vi "D+M Sense.vi"(8 "error in":errorcluster) -> (0 "error out":errorcluster, 2 "Result":string, 3 "RESULT":bool)   [LabVIEW 2021]
uses:
  DUT/DUT_Cmd.ctl
  10054_Control Folder/Support/10054_states.ctl
panel:
  out "Command Response 2":string
  out "number 2":dbl
  out "UnPlugged":bool
  out "Plugged":bool
  out "number":dbl
  out "Command Response":string
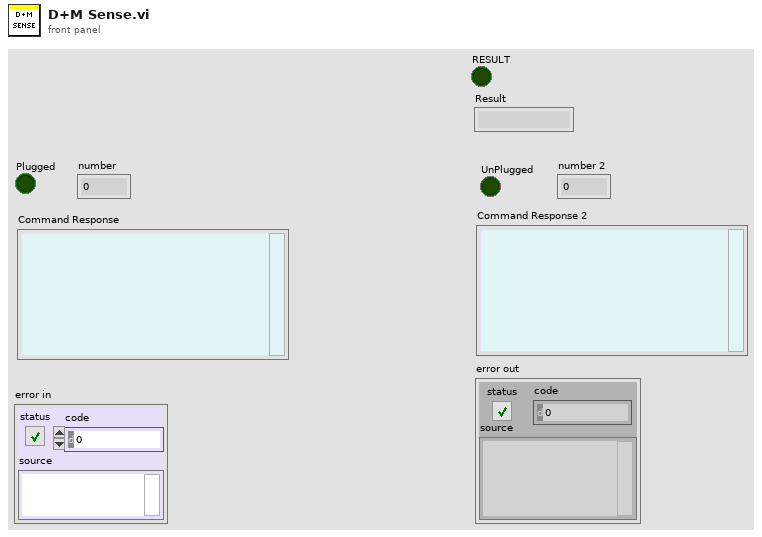
[diagram p1: front panel]
types:
  T1 = typedef "10054_states.ctl" = enum16{"Pilz-1", "Pilz-2", "AC CON - 2", "AC CON - 3", "AC CON - 4", "AC CON - 5", "Tower Lamp - Red", "Tower Lamp - Amber", "Tower Lamp - Green", "FAN 1 & 2", "FAN 3 & 4", "FAN 5 & 6", "Load - 1 10A", "Load - 2 10A", "Load - 3 5A", "Load - 4 5A", "Load - 5 2A", "TP49 - 12V", "TP20 - 5V", "TP148 - 3.3", "TP193 - GND", "J11.1 POS", "J11.2 NEG", "Noti LED POS", "Noti LED NEG", "Noti LED  5V", "D+M J14.1 - 3.3", "D+M J14.2 - GND", "NFC - 1", "NFC - 2"}
  T2 = typedef "DUT_Cmd.ctl" = enum16{"Unlock serial", "Stop console logs", "Release emergency at start", "Read firmware", "WiFi credentials", "WiFi connected", "WiFi SSID", "Board revision", "ADC_NTC_TEMP", "ADC_TYPE2_RCD_CURRENT", "PCBA serial write", "PCBA serial readback", "Start energy meter", "Energy meter Vac", "Energy meter Iac", "Energy meter PF", "Energy meter energy", "Provision", "Set gateway identity", "CP checklist", "Earth detect", "D+M sense unplugged", "D+M sense plugged", "Output relay weld", "Start diagnostics", "Relay 1 on", "Relay 2 on", "Emergency pressed", "Release emergency", "Emergency released", "Unlock serial for 5 A", "Board current (5 A)", "Unlock serial for 15 A", "Board current (15 A)", "Unlock serial for 0 A", "NFC tag", "Start diagnostics again", "Relay 2 off", "Relay 1 off", "End diagnostics", "Load current (5 A) [No USB station]", "Load current (15 A) [No USB station]", "Load current (0 A) [No USB station]", "NFC tag [No USB station]", "Battery Voltage", "FW Power reset", "Notification LED", "O/P Relay weld Detection", "Earth Detection", "12V ", "5V", "3.3V"}
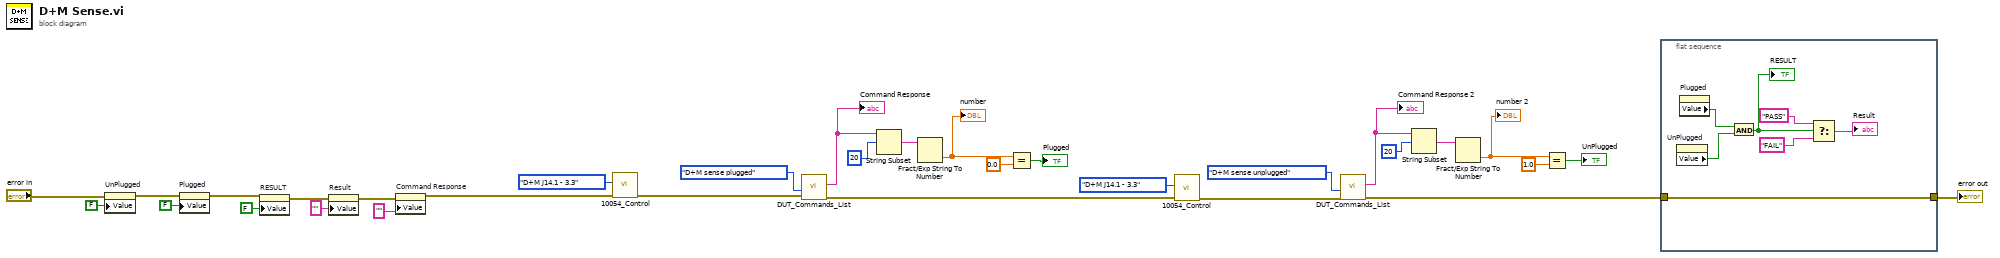
[diagram p0: block diagram]
diagram:
  n1 = property on="UnPlugged" class="Bool (strict)"(error in="error in", "Value"=FALSE ("UnPlugged")) -> (error out=w15:errorcluster)  [unwired: 1 in, 1 out]
  n2 = property on="Plugged" class="Bool (strict)"(error in=w15, "Value"=FALSE ("Plugged")) -> (error out=w14:errorcluster)  [unwired: 1 in, 1 out]
  n3 = property on="RESULT" class="Bool (strict)"(error in=w14, "Value"=FALSE ("RESULT")) -> (error out=w13:errorcluster)  [unwired: 1 in, 1 out]
  n4 = property on="Result" class="Str"(error in=w13, "Value"="" ("Result")) -> (error out=w12:errorcluster)  [unwired: 1 in, 1 out]
  n5 = property on="Command Response" class="Str"(error in=w12, "Value"="" ("Command Response")) -> (error out=w2:errorcluster)  [unwired: 1 in, 1 out]
  n6 = call "10054_Control.vi"("error in"=w2, "Pin"=10054_states."D+M J14.1 - 3.3") -> ("error out"=w1:errorcluster)  [unwired: 5 in, 3 out]
  n7 = call "DUT_Commands_List.vi"("error in"=w1, "DUT Cmd"=DUT_Cmd."D+M sense plugged") -> ("error out"=w6:errorcluster, "Command Response"=w30:string)  [unwired: 7 in, 1 out]
  "Command Response" <- w30
  n8 = String Subset(string=w30, offset (0)=20) -> (substring=w28:string)  [unwired: 1 in]
  n9 = Fract/Exp String To Number(string=w28) -> (number=w27:dbl)  [unwired: 3 in, 1 out]
  "number" <- w27
  n10 = Equal?(x=w27, y=0.0) -> (x = y?=→"Plugged":bool)
  n11 = call "10054_Control.vi"("error in"=w6, "Pin"=10054_states."D+M J14.1 - 3.3") -> ("error out"=w5:errorcluster)  [unwired: 5 in, 3 out]
  n12 = call "DUT_Commands_List.vi"("error in"=w5, "DUT Cmd"=DUT_Cmd."D+M sense unplugged") -> ("error out"=w17:errorcluster, "Command Response"=w19:string)  [unwired: 7 in, 1 out]
  "Command Response 2" <- w19
  n13 = String Subset(string=w19, offset (0)=20) -> (substring=w21:string)  [unwired: 1 in]
  n14 = Fract/Exp String To Number(string=w21) -> (number=w22:dbl)  [unwired: 3 in, 1 out]
  "number 2" <- w22
  n15 = Equal?(x=w22, y=1.0) -> (x = y?=→"UnPlugged":bool)
  n16 = flat-sequence {
    tunnel: w17 -> [w34]
    tunnel: [w34] -> w16
    frame #0 {
      n17 = property on="UnPlugged" class="Bool (strict)"() -> ("Value"=w35:bool)  [unwired: 2 in, 2 out]
      n18 = property on="Plugged" class="Bool (strict)"() -> ("Value"=w36:bool)  [unwired: 2 in, 2 out]
      n19 = And(x=w36, y=w35) -> (x .and. y?=w33:bool)
      "RESULT" <- w33
      n20 = Select(t="PASS", s=w33, f="FAIL") -> (s? t:f=→"Result":string)
    }
  }
  "error out" <- w16
